vi "PropertyAdd.vi"(8 "error in":errorcluster, 11 "Data":T4) -> (0 "error out":errorcluster, 3 "Data 2":T4)   [LabVIEW 2017]
doc: "<B>This VI is used for adding a new property to the Caps file.</B>"
uses:
  Ctrl/Data.ctl
  Ctrl/Caps.ctl
  Ctrl/Property.ctl
  Ctrl/PhysicalChannel.ctl
  Ctrl/Register.ctl
  Ctrl/Bitfield.ctl
  Ctrl/Scale.ctl
  Ctrl/ScaleType.ctl
  Ctrl/Enum.ctl
  Ctrl/EnumValue.ctl
  Ctrl/Type Tab.ctl
  Ctrl/UserInput.ctl
  Ctrl/compond commands.ctl
panel:
  out "Data Range":T1
  in  "Min(Double)":dbl
  in  "Max(Double)":dbl
  in  "Max(U64)":u64
  in  "Min(U64)":u64
  in  "Min(I64)":i64
  in  "Max(I64)":i64
  in  "Max(U32)":u32
  in  "Min(U32)":u32
  in  "Min(I32)":i32
  in  "Max(I32)":i32
  in  "NewPropertyParameter:":T2 {"Value_Cluster"."U8" format="%.0x"; "Value_Cluster"."Ring" items=["False", "True"]; "Value_Cluster"."DBL" format="%#_16g"; "Scale" items=["NoScale"]; "Access" items=["Read Only", "Write Only", "Read/Write"]; "Bitfield" items=["Version/Timestamp", "TemperatureThreshold/TempThrehold", "TemperatureRegister3/AcquiredTemperature", "TemperatureRegister1/AcquiredTemperature", "TemperatureRegister2/AcquiredTemperature", "TemperatureRegister0/AcquiredTemperature", "Status/FlashWriteProtect", "Status/FlashHold", "Status/ClearWriteDuringUpdateError", "Status/SlscInterfaceUnusedPin", "Status/StrapOption", "Status/PowerGood5V", "Status/PowerGood24V", "Status/BoardFault", "Status/WriteDuringUpdateError", "Status/UpdateDone", "ClearFaults/OverTemperatureDigital", "ClearFaults/OverTemperature", "ClearFaults/OverCurrentOnBus", "ClearFaults/OverCurrentLow", "ClearFaults/OverCurrentHigh", "DigitalTempertureFault/TempFaultVector", "OverTemperature/OvertemperatureDifferential", "OverTemperature/OvertemperatureChannel", "OvercurrentLowStatus/OvercurrentLow", "OvercurrentHighStatus/OvercurrentHigh", "OvercurrentOnBus/BusB_OverCurrent", "OvercurrentOnBus/BusA_OverCurrent", "UpdateRegister/Update", "BoardControl/UpdateModeField", "BoardControl/BoardEnable", "BoardControl/TempSensorEnable", "StateRegister7/ChannelConnect", "StateRegister7/BusSelectionM", "StateRegister7/LoadEnableM", "StateRegister7/BusSelectionP", "StateRegister7/LoadEnableP", "PreloadRegister7/ChannelConnect", "PreloadRegister7/BusSelectionM", "PreloadRegister7/LoadEnableM", "PreloadRegister7/BusSelectionP", "PreloadRegister7/LoadEnableP", "StateRegister6/ChannelConnect", "StateRegister6/BusSelectionM", "StateRegister6/LoadEnableM", "StateRegister6/BusSelectionP", "StateRegister6/LoadEnableP", "PreloadRegister6/ChannelConnect", "PreloadRegister6/BusSelectionM", "PreloadRegister6/LoadEnableM", "PreloadRegister6/BusSelectionP", "PreloadRegister6/LoadEnableP", "StateRegister5/ChannelConnect", "StateRegister5/BusSelectionM", "StateRegister5/LoadEnableM", "StateRegister5/BusSelectionP", "StateRegister5/LoadEnableP", "PreloadRegister5/ChannelConnect", "PreloadRegister5/BusSelectionM", "PreloadRegister5/LoadEnableM", "PreloadRegister5/BusSelectionP", "PreloadRegister5/LoadEnableP", "StateRegister4/ChannelConnect", "StateRegister4/BusSelectionM", "StateRegister4/LoadEnableM", "StateRegister4/BusSelectionP", "StateRegister4/LoadEnableP", "PreloadRegister4/ChannelConnect", "PreloadRegister4/BusSelectionM", "PreloadRegister4/LoadEnableM", "PreloadRegister4/BusSelectionP", "PreloadRegister4/LoadEnableP", "StateRegister3/ChannelConnect", "StateRegister3/BusSelectionM", "StateRegister3/LoadEnableM", "StateRegister3/BusSelectionP", "StateRegister3/LoadEnableP", "PreloadRegister3/ChannelConnect", "PreloadRegister3/BusSelectionM", "PreloadRegister3/LoadEnableM", "PreloadRegister3/BusSelectionP", "PreloadRegister3/LoadEnableP", "StateRegister2/ChannelConnect", "StateRegister2/BusSelectionM", "StateRegister2/LoadEnableM", "StateRegister2/BusSelectionP", "StateRegister2/LoadEnableP", "PreloadRegister2/ChannelConnect", "PreloadRegister2/BusSelectionM", "PreloadRegister2/LoadEnableM", "PreloadRegister2/BusSelectionP", "PreloadRegister2/LoadEnableP", "StateRegister1/ChannelConnect", "StateRegister1/BusSelectionM", "StateRegister1/LoadEnableM", "StateRegister1/BusSelectionP", "StateRegister1/LoadEnableP", "PreloadRegister1/ChannelConnect", "PreloadRegister1/BusSelectionM", "PreloadRegister1/LoadEnableM", "PreloadRegister1/BusSelectionP", "PreloadRegister1/LoadEnableP", "StateRegister0/ChannelConnect", "StateRegister0/BusSelectionM", "StateRegister0/LoadEnableM", "StateRegister0/BusSelectionP", "StateRegister0/LoadEnableP", "PreloadRegister0/ChannelConnect", "PreloadRegister0/BusSelectionM", "PreloadRegister0/LoadEnableM", "PreloadRegister0/BusSelectionP", "PreloadRegister0/LoadEnableP", "SlowFilterCount/SlowCount", "FastFilterCount/FastCount", "SwitchDelayTime/CycleDelays", "InterruptAck/DigitalOverTemperatureIntAck", "InterruptAck/OverTemperatureIntAck", "InterruptAck/OverCurrentOnBusIntAck", "InterruptAck/OverCurrentLowIntAck", "InterruptAck/OverCurrentHighIntAck", "InterruptAck/UpdateDoneAck", "InterruptDisable/DigitalOverTemperatureIntDisable", "InterruptDisable/OverTemperatureIntDisable", "InterruptDisable/OverCurrentOnBusIntDisable", "InterruptDisable/OverCurrentLowIntDisable", "InterruptDisable/OverCurrentHighIntDisable", "InterruptDisable/UpdateDoneDisable", "InterruptEnable/DigitalOverTemperatureIntEnable", "InterruptEnable/OverTemperatureIntEnable", "InterruptEnable/OverCurrentOnBusIntEnable", "InterruptEnable/OverCurrentLowIntEnable", "InterruptEnable/OverCurrentHighIntEnable", "InterruptEnable/UpdateDoneEnable", "InterruptMask/DigitalOverTemperatureIntMask", "InterruptMask/OverTemperatureIntMask", "InterruptMask/OverCurrentOnBusIntMask", "InterruptMask/OverCurrentLowIntMask", "InterruptMask/OverCurrentHighIntMask", "InterruptMask/UpdateDoneMask", "InterruptStatus/DigitalOverTemperatureIntStatus", "InterruptStatus/OverTemperatureIntStatus", "InterruptStatus/OverCurrentOnBusIntStatus", "InterruptStatus/OverCurrentLowIntStatus", "InterruptStatus/OverCurrentHighIntStatus", "InterruptStatus/UpdateDone"]}
  out "CurrentAddPosition:":string="Current Adding Position:  NI.DateCode"
  in  "User Input":T3
  # "Value"
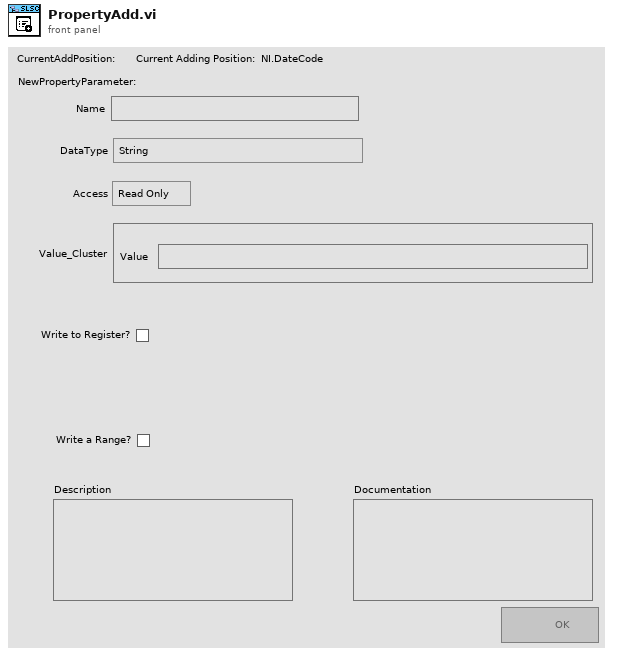
[diagram p1: front panel]
types:
  T1 = typedef "Type Tab.ctl" = enum32{"String", "Double", "U64", "I64", "U32", "I32", "Bool"}
  T2 = cluster{"Name":string, "DataType":enum16{"String", "Double", "U64", "I64", "U32", "I32", "Bool"}, "Bitfield":u16, "Access":u16, "Description":string, "Documentation":string, "OK Button":bool, "Scale":u16, "Write a Register?":bool, "Write a Range?":bool, "Value_Cluster":cluster{"DBL":dbl, "Ring":u16, "I64":i64, "U64":u64, "I32":i32, "U32":u32, "I8":i8, "U8":u8, "String":string}}
  T3 = typedef "UserInput.ctl" = cluster{"NewPropertyParameter":cluster{"Name":string, "DataType":enum16{"String", "Double", "U64", "I64", "U32", "I32", "Bool"}, "Bitfield":u16, "Access":u16, "Description":string, "Documentation":string, "OK Button":bool, "Scale method":u16, "Write a Register?":bool, "Write a Range?":bool, "Value_Cluster":cluster{"DBL":dbl, "Ring":u16, "I64":i64, "U64":u64, "I32":i32, "U32":u32, "I8":i8, "U8":u8, "String":string}}, "Min_Max_Cluster":cluster{"Min(Double)":dbl, "Max(Double)":dbl, "Min(U64)":u64, "Max(U64)":u64, "Min(I64)":i64, "Max(I64)":i64, "Min(U32)":u32, "Max(U32)":u32, "Min(I32)":i32, "Max(I32)":i32}, "Scale method":string, "Access":string, "Bitfield":string}
  T4 = typedef "Data.ctl" = cluster{"Ref Cluster":cluster{"String":refnum<vi>, "U8":refnum<vi>, "I8":refnum<vi>, "U32":refnum<vi>, "I32":refnum<vi>, "U64":refnum<vi>, "I64":refnum<vi>, "Ring":refnum<vi>, "DBL":refnum<vi>, "Add":refnum<vi>, "Remove":refnum<vi>, "Property tree":refnum<vi>, "confirm":refnum<vi>}, "JSON Text":string, "Original JSON Text":string, "Caps":T5, "SLSC Output Tree":cluster{"Left Cell String":string, "Child Text":string[], "Child Tag":string, "Item Indent":i32, "Child Only?":bool, "Glyph Index":i32, "offline value":variant}[], "Ref Index and Control Type":cluster{"index":i32, "Datatype":string}, "Selected Type and name":cluster{"Selected Type":enum16{"Property", "Physical Channel", "Other"}, "Selected Property Name":string}, "Update whole Tree?":bool}
  T5 = typedef "Caps.ctl" = cluster{"properties":T6[], "physical channels":T7[], "registers":T8[], "scales":T10[], "enums":T12[], "productName":string}
  T6 = typedef "Property.ctl" = cluster{"name":string, "bitfield":string, "value":variant, "dataType":string, "min":variant, "max":variant, "scale":string, "access":string}
  T7 = typedef "PhysicalChannel.ctl" = cluster{"name":string, "properties":T6[]}
  T8 = typedef "Register.ctl" = cluster{"name":string, "address":i32, "size":i32, "bitfields":T9[], "initialValue":variant, "connectedProperties":string[]}
  T9 = typedef "Bitfield.ctl" = cluster{"name":string, "offset":i32, "size":i32, "signed":bool}
  T10 = typedef "Scale.ctl" = cluster{"name":string, "type":T11, "params":variant}
  T11 = typedef "ScaleType.ctl" = enum16{"NoScale", "Table", "Polynomial", "Linear"}
  T12 = typedef "Enum.ctl" = cluster{"name":string, "values":T13[]}
  T13 = typedef "EnumValue.ctl" = cluster{"name":string, "value":i32}
  T14 = cluster{"Min(Double)":dbl, "Max(Double)":dbl, "Min(U64)":u64, "Max(U64)":u64, "Min(I64)":i64, "Max(I64)":i64, "Min(U32)":u32, "Max(U32)":u32, "Min(I32)":i32, "Max(I32)":i32}
  T15 = enum16{"String", "Double", "U64", "I64", "U32", "I32", "Bool"}
  T16 = enum8{"Enabled", "Disabled", "Disabled and Grayed Out"}
  T17 = cluster{"Name":string, "DataType":enum16{"String", "Double", "U64", "I64", "U32", "I32", "Bool"}, "Bitfield":u16, "Access":u16, "Description":string, "Documentation":string, "OK Button":bool, "Scale method":u16, "Write a Register?":bool, "Write a Range?":bool, "Value_Cluster":cluster{"DBL":dbl, "Ring":u16, "I64":i64, "U64":u64, "I32":i32, "U32":u32, "I8":i8, "U8":u8, "String":string}}
  T18 = cluster{"Duplicated?":bool, "InRange?":bool, "IsEmpty?":bool}
  T19 = typedef "compond commands.ctl" = enum16{"Get Property Array", "Get Physical Channel Property Array", "Get the Selected Position", "Get Property and Physical Channel Name", "Get Type and Value", "Make and Set a new Property", "Modify the Value", "Delete a Property"}
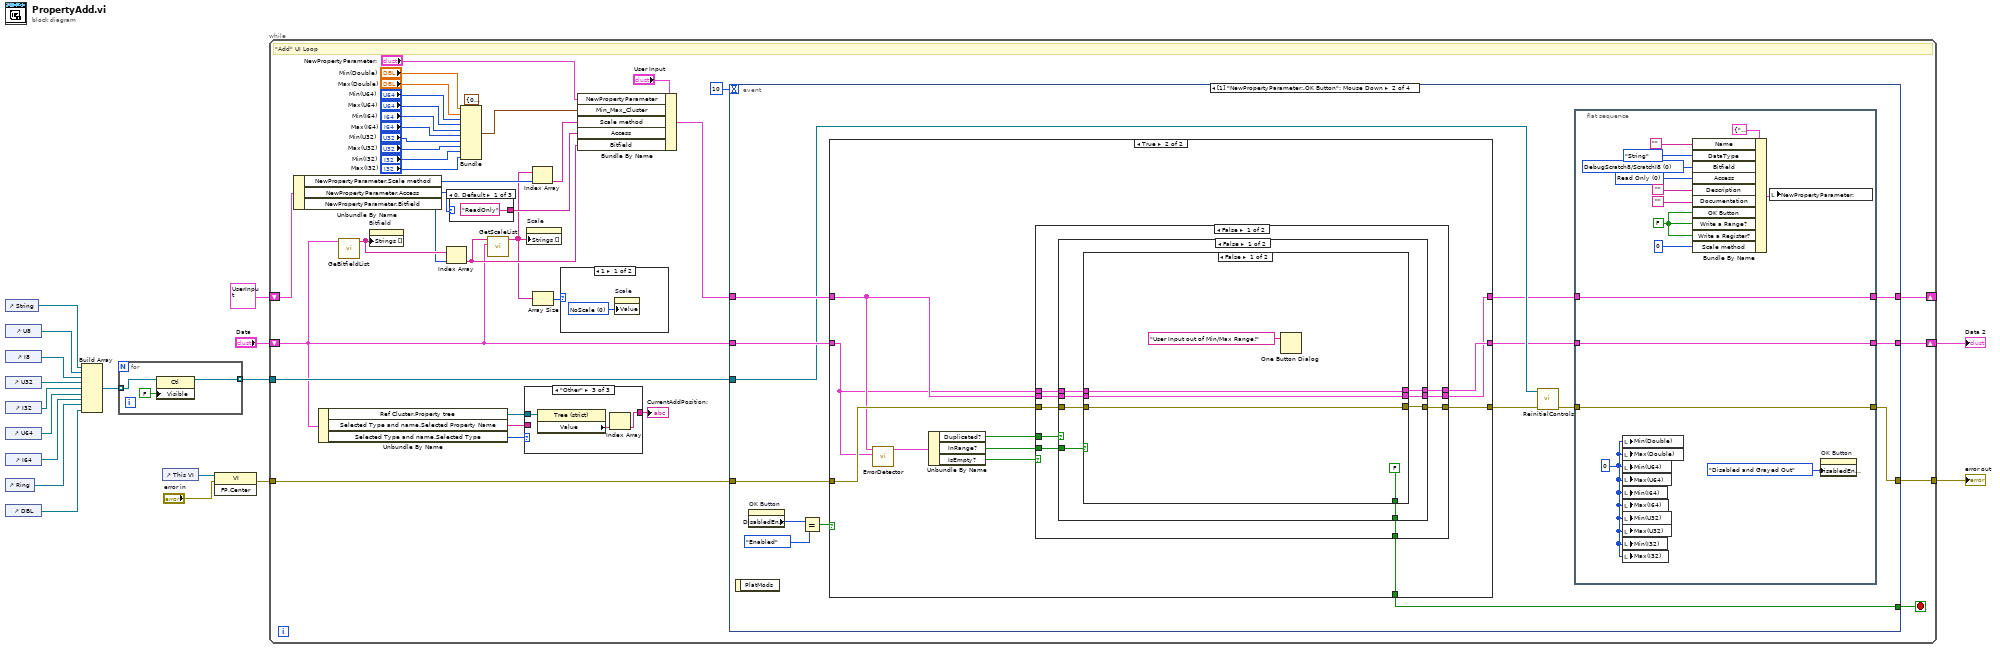
[diagram p0: block diagram]
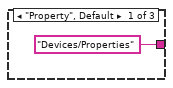
[diagram p2: hidden frame]
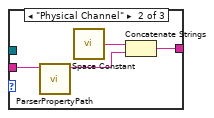
[diagram p3: hidden frame]
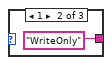
[diagram p5: hidden frame]
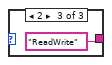
[diagram p6: hidden frame]
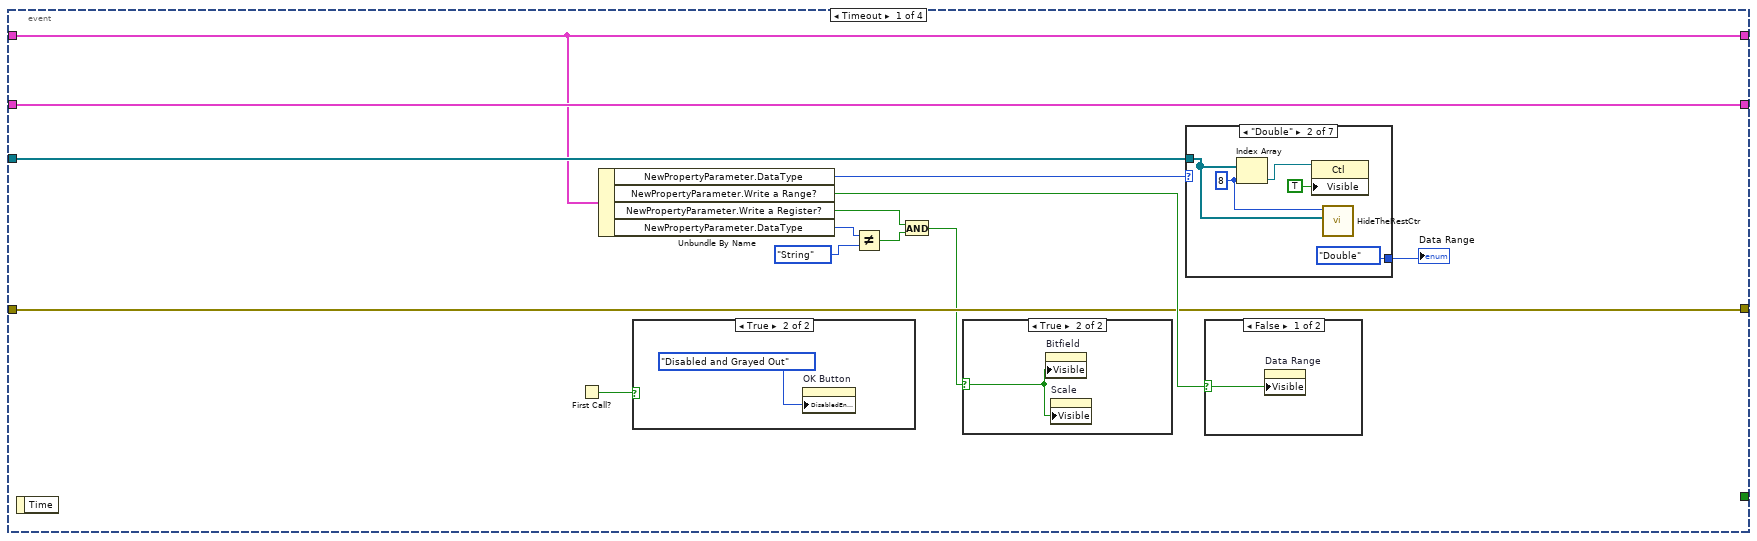
[diagram p7: hidden frame]
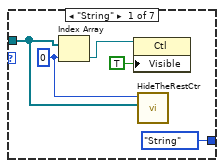
[diagram p8: hidden frame]
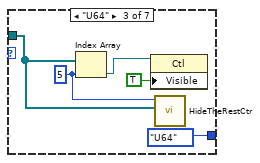
[diagram p9: hidden frame]
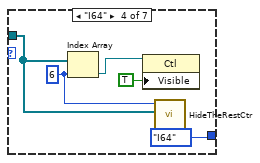
[diagram p10: hidden frame]
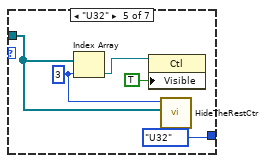
[diagram p11: hidden frame]
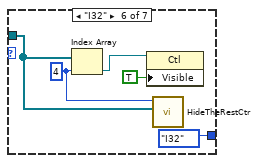
[diagram p12: hidden frame]
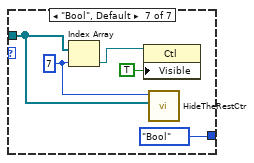
[diagram p13: hidden frame]
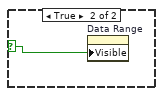
[diagram p14: hidden frame]
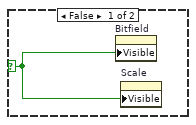
[diagram p15: hidden frame]
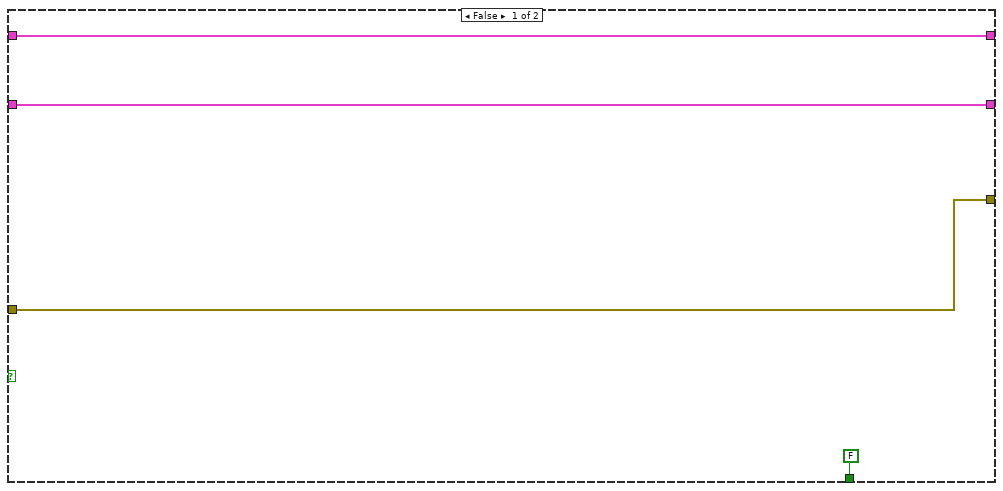
[diagram p17: hidden frame]
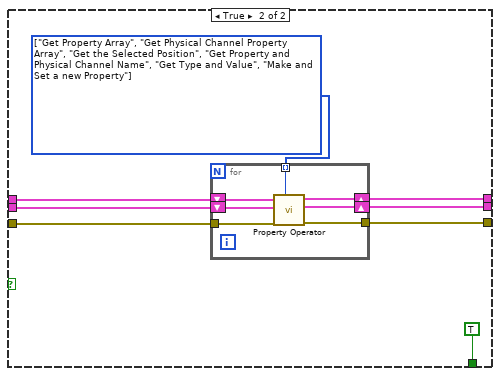
[diagram p18: hidden frame]
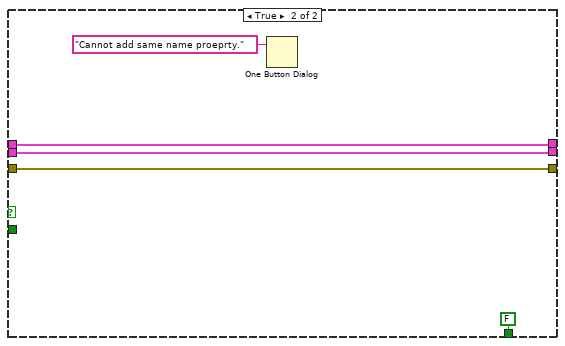
[diagram p19: hidden frame]
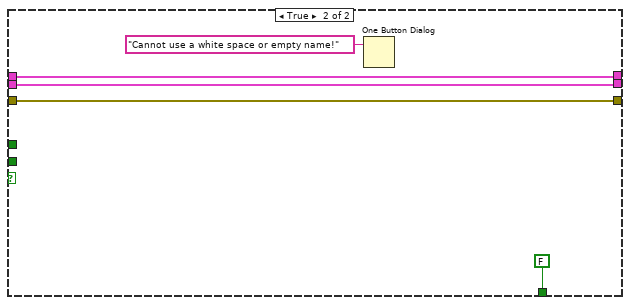
[diagram p20: hidden frame]
diagram:
  n1 = control-ref of="String"() -> (w18:refnum<vi>)
  n2 = control-ref of="U8"() -> (w17:refnum<vi>)
  n3 = control-ref of="I8"() -> (w16:refnum<vi>)
  n4 = control-ref of="U32"() -> (w15:refnum<vi>)
  n5 = control-ref of="I32"() -> (w14:refnum<vi>)
  n6 = control-ref of="U64"() -> (w13:refnum<vi>)
  n7 = control-ref of="I64"() -> (w12:refnum<vi>)
  n8 = control-ref of="Ring"() -> (w11:refnum<vi>)
  n9 = control-ref of="DBL"() -> (w10:refnum<vi>)
  n10 = Build Array(w18, w17, w16, w15, w14, w13, w12, w11, w10) -> (w3:refnum<vi>[])
  n11 = for {
    tunnel: w3 -> [w21] mode=indexing
    tunnel: [w19] -> w2 mode=indexing
    n12 = property class="Ctl"(reference=w21, "Visible"=FALSE) -> (reference out=w19:refnum<vi>)  [unwired: 1 in, 1 out]
  }
  n13 = control-ref of="This VI"() -> (w6:refnum<vi>)
  n14 = invoke class="VI" method="FP.Center"(reference=w6, error in="error in") -> (error out=w5:errorcluster)  [unwired: 1 in, 2 out]
  n15 = while {
    tunnel: w5 -> [w53]
    tunnel: [w57] -> w9
    shift-right: [w58] -> w7
    shift-left: "Data" -> [w26]
    shift-right: [w30] -> _
    shift-left: T3 {"NewPropertyParameter"={"Name"="", "DataType"=enum."String", "Bitfield"=0, "Access"=0, "Description"="", "Documentation"="", "OK Button"=FALSE, "Scale method"=0, "Write a Register?"=FALSE, "Write a Range?"=FALSE, "Value_Cluster"={"DBL"=0.0, "Ring"=0, "I64"=0, "U64"=0, "I32"=0, "U32"=0, "I8"=0, "U8"=0, "String"=""}}, "Min_Max_Cluster"={"Min(Double)"=0.0, "Max(Double)"=0.0, "Min(U64)"=0, "Max(U64)"=0, "Min(I64)"=0, "Max(I64)"=0, "Min(U32)"=0, "Max(U32)"=0, "Min(I32)"=0, "Max(I32)"=0}, "Scale method"="", "Access"="", "Bitfield"=""} ("User Input") -> [w40]
    tunnel: w2 -> [w31]
    stop <- w54 stop-if-true
    # "\"Add\" UI Loop"
    n16 = Unbundle By Name(w40) -> ("NewPropertyParameter.Scale method"=w36:u16, "NewPropertyParameter.Access"=w37:u16, "NewPropertyParameter.Bitfield"=w38:u16)
    n17 = Unbundle By Name(w26) -> ("Ref Cluster.Property tree"=w23:refnum<vi>, "Selected Type and name.Selected Property Name"=w25:string, "Selected Type and name.Selected Type"=w24:enum16{"Property", "Physical Channel", "Other"})
    n18 = call "GeBitfieldList.vi"("Data"=w26) -> ("Array"=w39:string[])  [unwired: 10 in]
    n19 = property on="Bitfield" class="Ring (strict)"("Strings []"=w39) -> ()  [unwired: 2 in, 2 out]
    n20 = Index Array(array=w39, index=w38) -> (element=w34:string)
    n21 = case shown="0, Default" w37 {
      tunnel: ["ReadOnly" "WriteOnly" "ReadWrite"] -> w33
      frame 0, Default {
      }
      frame 1 {
      }
      frame 2 {
      }
    }
    n22 = Bundle(cluster=T14 {"Min(Double)"=0.0, "Max(Double)"=0.0, "Min(U64)"=0, "Max(U64)"=0, "Min(I64)"=0, "Max(I64)"=0, "Min(U32)"=0, "Max(U32)"=0, "Min(I32)"=0, "Max(I32)"=0} ("Min_Max_Cluster"), "Min(Double)"="Min(Double)", "Max(Double)"="Max(Double)", "Min(U64)"="Min(U64)", "Max(U64)"="Max(U64)", "Min(I64)"="Min(I64)", "Max(I64)"="Max(I64)", "Min(U32)"="Min(U32)", "Max(U32)"="Max(U32)", "Min(I32)"="Min(I32)", "Max(I32)"="Max(I32)") -> (w52:T14)
    n23 = call "GetScaleList.vi"("Data in"=w26, "Bitfield in"=w34) -> ("output array"=w32:string[])  [unwired: 9 in]
    n24 = case shown="\"Other\"" w24 {
      tunnel: ["Devices/Properties" w63 w64] -> w28
      tunnel: w25 -> [_ w61 _]
      tunnel: w23 -> [_ _ w66]
      frame "Property", Default {
      }
      frame "Physical Channel" {
        n25 = call "ParserPropertyPath.vi"("Seleted Item Name"=w61) -> ("Physical channel"=w60:string)  [unwired: 7 in, 1 out]
        n26 = call <vilib>:"Space Constant.vi"() -> ("String"=w62:string)
        n27 = Concatenate Strings(w62, w60) -> (w63:string)
      }
      frame "Other" {
        n28 = property class="Tree (strict)"(reference=w66) -> ("Value"=w65:string[])  [unwired: 1 in, 2 out]
        n29 = Index Array(array=w65) -> (element=w64:string)  [unwired: 1 in]
      }
    }
    "CurrentAddPosition:" <- w28
    n30 = property on="Scale" class="Ring (strict)"("Strings []"=w32) -> ()  [unwired: 2 in, 2 out]
    n31 = Index Array(array=w32, index=w36) -> (element=w35:string)
    n32 = Array Size(array=w32) -> (size(s)=w55:i32)
    n33 = case shown="1" w55 {
      frame 1 {
        w67 = u16 0 items=["NoScale"] ("Scale method")
        n34 = property on="Scale" class="Ring (strict)"("Value"=w67) -> ()  [unwired: 2 in, 2 out]
      }
      frame Default {
      }
    }
    n35 = Bundle By Name(cluster="User Input", "NewPropertyParameter"="NewPropertyParameter:", "Min_Max_Cluster"=w52, "Scale method"=w35, "Access"=w33, "Bitfield"=w34) -> (w27:T3)
    n36 = event shown="[1] \"NewPropertyParameter:.OK Button\": Mouse Down" {
      selector: _ -> [_ _ _ _]
      dyn-events: _ -> [_ _ _ _]
      timeout: 10 -> [_ _ _ _]
      tunnel: w26 -> [w81 w138 w219 w236]
      tunnel: [w81 w127 w219 w236] -> w58
      tunnel: [w77 w124 w216 w235] -> w57
      tunnel: [_ w133 _ TRUE] -> w54
      tunnel: w53 -> [w77 w132 w216 w232]
      tunnel: w31 -> [w78 w130 _ w231]
      tunnel: w27 -> [w76 w131 w217 w230]
      tunnel: [w76 w125 w217 w230] -> w30
      event Timeout {
        n37 = event-data() -> ()  [unwired: 1 in, 1 out]
        n38 = First Call?() -> (First Call?: T/F=w82:bool)
        n39 = Unbundle By Name(w76) -> ("NewPropertyParameter.DataType"=w80:T15, "NewPropertyParameter.Write a Range?"=w79:bool, "NewPropertyParameter.Write a Register?"=w72:bool, "NewPropertyParameter.DataType"=w75:T15)
        n40 = case shown="True" w82 {
          frame False {
          }
          frame True {
            n41 = property on="OK Button" class="Bool (strict)"("DisabledEnum"=T16."Disabled and Grayed Out" ("Disabled")) -> ()  [unwired: 2 in, 2 out]
          }
        }
        n42 = Not Equal?(x=w75, y=T15."String") -> (x != y?=w73:bool)
        n43 = And(x=w72, y=w73) -> (x .and. y?=w71:bool)
        n44 = case shown="True" w71 {
          selector: w71 -> [w121 w122]
          frame False {
            n45 = property on="Bitfield" class="Ring (strict)"("Visible"=w121) -> ()  [unwired: 2 in, 2 out]
            n46 = property on="Scale" class="Ring (strict)"("Visible"=w121) -> ()  [unwired: 2 in, 2 out]
          }
          frame True {
            n47 = property on="Bitfield" class="Ring (strict)"("Visible"=w122) -> ()  [unwired: 2 in, 2 out]
            n48 = property on="Scale" class="Ring (strict)"("Visible"=w122) -> ()  [unwired: 2 in, 2 out]
          }
        }
        n49 = case shown="\"Double\"" w80 {
          tunnel: [Type_Tab."String" ("Tab Control") Type_Tab."Double" ("Tab Control") Type_Tab."U64" ("Tab Control") Type_Tab."I64" ("Tab Control") Type_Tab."U32" ("Tab Control") Type_Tab."I32" ("Tab Control") Type_Tab."Bool" ("Tab Control")] -> w83
          tunnel: w78 -> [w84 w89 w94 w99 w104 w109 w114]
          frame "String" {
            w87 = 0 ("index")
            n50 = Index Array(array=w84, index=w87) -> (element=w85:refnum<vi>)
            n51 = property class="Ctl"(reference=w85, "Visible"=TRUE) -> ()  [unwired: 1 in, 2 out]
            n52 = call "HideTheRestCtr.vi"("Array"=w84, "index"=w87) -> ()  [unwired: 10 in]
          }
          frame "Double" {
            w92 = 8 ("index")
            n53 = Index Array(array=w89, index=w92) -> (element=w90:refnum<vi>)
            n54 = property class="Ctl"(reference=w90, "Visible"=TRUE) -> ()  [unwired: 1 in, 2 out]
            n55 = call "HideTheRestCtr.vi"("Array"=w89, "index"=w92) -> ()  [unwired: 10 in]
          }
          frame "U64" {
            w97 = 5 ("index")
            n56 = Index Array(array=w94, index=w97) -> (element=w95:refnum<vi>)
            n57 = property class="Ctl"(reference=w95, "Visible"=TRUE) -> ()  [unwired: 1 in, 2 out]
            n58 = call "HideTheRestCtr.vi"("Array"=w94, "index"=w97) -> ()  [unwired: 10 in]
          }
          frame "I64" {
            w102 = 6 ("index")
            n59 = Index Array(array=w99, index=w102) -> (element=w100:refnum<vi>)
            n60 = property class="Ctl"(reference=w100, "Visible"=TRUE) -> ()  [unwired: 1 in, 2 out]
            n61 = call "HideTheRestCtr.vi"("Array"=w99, "index"=w102) -> ()  [unwired: 10 in]
          }
          frame "U32" {
            w107 = 3 ("index")
            n62 = Index Array(array=w104, index=w107) -> (element=w105:refnum<vi>)
            n63 = property class="Ctl"(reference=w105, "Visible"=TRUE) -> ()  [unwired: 1 in, 2 out]
            n64 = call "HideTheRestCtr.vi"("Array"=w104, "index"=w107) -> ()  [unwired: 10 in]
          }
          frame "I32" {
            w112 = 4 ("index")
            n65 = Index Array(array=w109, index=w112) -> (element=w110:refnum<vi>)
            n66 = property class="Ctl"(reference=w110, "Visible"=TRUE) -> ()  [unwired: 1 in, 2 out]
            n67 = call "HideTheRestCtr.vi"("Array"=w109, "index"=w112) -> ()  [unwired: 10 in]
          }
          frame "Bool", Default {
            w117 = 7 ("index")
            n68 = Index Array(array=w114, index=w117) -> (element=w115:refnum<vi>)
            n69 = property class="Ctl"(reference=w115, "Visible"=TRUE) -> ()  [unwired: 1 in, 2 out]
            n70 = call "HideTheRestCtr.vi"("Array"=w114, "index"=w117) -> ()  [unwired: 10 in]
          }
        }
        "Data Range" <- w83
        n71 = case shown="False" w79 {
          selector: w79 -> [w119 w120]
          frame False {
            n72 = property on="Data Range" class="TabCtl (strict)"("Visible"=w119) -> ()  [unwired: 2 in, 2 out]
          }
          frame True {
            n73 = property on="Data Range" class="TabCtl (strict)"("Visible"=w120) -> ()  [unwired: 2 in, 2 out]
          }
        }
      }
      event "NewPropertyParameter:.OK Button": Mouse Down {
        n74 = event-data() -> ()  [unwired: 1 in, 1 out]
        n75 = property on="OK Button" class="Bool (strict)"() -> ("DisabledEnum"=w135:T16)  [unwired: 2 in, 2 out]
        n76 = Equal?(x=w135, y=T16."Enabled") -> (x = y?=w136:bool)
        n77 = case shown="True" w136 {
          tunnel: w138 -> [w157 w162]
          tunnel: [w157 w167] -> w128
          tunnel: [w155 w166] -> w137
          tunnel: [FALSE w168] -> w133
          tunnel: w131 -> [w154 w163]
          tunnel: w132 -> [w155 w165]
          tunnel: [w154 w164] -> w126
          frame False {
          }
          frame True {
            n78 = call "ErrorDetector.vi"("Data"=w162, "User Input"=w163) -> ("Cluster"=w161:T18)  [unwired: 9 in]
            n79 = Unbundle By Name(w161) -> ("Duplicated?"=w160:bool, "InRange?"=w159:bool, "IsEmpty?"=w158:bool)
            n80 = case shown="False" w158 {
              tunnel: [w177 FALSE] -> w168
              tunnel: [w176 w213] -> w167
              tunnel: [w175 w214] -> w166
              tunnel: w165 -> [w174 w214]
              tunnel: [w173 w212] -> w164
              tunnel: w160 -> [w172 _]
              tunnel: w162 -> [w171 w213]
              tunnel: w159 -> [w170 _]
              tunnel: w163 -> [w169 w212]
              frame False {
                n81 = case shown="False" w172 {
                  tunnel: [w185 FALSE] -> w177
                  tunnel: [w184 w210] -> w176
                  tunnel: [w183 w208] -> w175
                  tunnel: w174 -> [w182 w208]
                  tunnel: [w181 w209] -> w173
                  tunnel: w169 -> [w180 w209]
                  tunnel: w171 -> [w179 w210]
                  tunnel: w170 -> [w178 _]
                  frame False {
                    n82 = case shown="False" w178 {
                      tunnel: [FALSE TRUE] -> w185
                      tunnel: w179 -> [w190 w197]
                      tunnel: [w190 w196] -> w184
                      tunnel: w180 -> [w189 w195]
                      tunnel: [w189 w194] -> w181
                      tunnel: w182 -> [w188 w193]
                      tunnel: [w188 w192] -> w183
                      frame False {
                        n83 = One Button Dialog(message="User Input out of Min/Max Range!") -> ()  [unwired: 1 in, 1 out]
                      }
                      frame True {
                        w191 = T19[] [enum."Get Property Array", enum."Get Physical Channel Property Array", enum."Get the Selected Position", enum."Get Property and Physical Channel Name", enum."Get Type and Value", enum."Make and Set a new Property"] items=["Get Property Array", "Get Physical Channel Property Array", "Get the Selected Position", "Get Property and Physical Channel Name", "Get Type and Value", "Make and Set a new Property", "Modify the Value", "Delete a Property"]
                        n84 = for {
                          tunnel: w193 -> [w201]
                          tunnel: [w200] -> w192
                          shift-right: [w204] -> w196
                          shift-left: w197 -> [w205]
                          shift-right: [w202] -> w194
                          shift-left: w195 -> [w203]
                          tunnel: w191 -> [w199] mode=indexing
                          n85 = call "Property Operator.vi"("Command"=w199, "error in"=w201, "User Input"=w203, "Data Input"=w205) -> ("error out"=w200:errorcluster, "User Input 2"=w202:T3, "Data Output"=w204:T4)  [unwired: 5 in]
                        }
                      }
                    }
                  }
                  frame True {
                    n86 = One Button Dialog(message="Cannot add same name proeprty.") -> ()  [unwired: 1 in, 1 out]
                  }
                }
              }
              frame True {
                n87 = One Button Dialog(message="Cannot use a white space or empty name!") -> ()  [unwired: 1 in, 1 out]
              }
            }
          }
        }
        n88 = call "ReinitialControls.vi"("error in (no error)"=w137, "Control reference Array"=w130) -> ("error out"=w129:errorcluster)  [unwired: 9 in]
        n89 = flat-sequence {
          tunnel: w129 -> [w144]
          tunnel: [w144] -> w124
          tunnel: w128 -> [w143]
          tunnel: [w143] -> w127
          tunnel: [w142] -> w125
          tunnel: w126 -> [w142]
          frame #0 {
            w141 = FALSE ("OK Button")
            w147 = u16 0 items=["Read Only", "Write Only", "Read/Write"] ("Access")
            w148 = u16 0 items=["DebugScratch8/ScratchI8", "DebugScratch8/Scratch8", "DebugScratch8/ScratchBool", "DebugScratch16/ScratchBool", "DebugScratch16/ScratchI8", "DebugScratch16/Scratch8", "DebugScratch16/ScratchI16", "DebugScratch16/Scratch16", "DebugScratch32/ScratchBool", "DebugScratch32/ScratchI8", "DebugScratch32/Scratch8", "DebugScratch32/ScratchI16", "DebugScratch32/Scratch16", "DebugScratch32/ScratchI32", "DebugScratch32/Scratch32", "DebugLeds/DebugLed3", "DebugLeds/DebugLed2", "DebugLeds/DebugLed1", "DebugLeds/DebugLed0", "DebugDipSwitch/DipSwitch8", "DebugDipSwitch/DipSwitch7", "DebugDipSwitch/DipSwitch6", "DebugDipSwitch/DipSwitch5", "DebugDipSwitch/DipSwitch4", "DebugDipSwitch/DipSwitch3", "DebugDipSwitch/DipSwitch2", "DebugDipSwitch/DipSwitch1", "DebugScratch64/ScratchBool", "DebugScratch64/ScratchI8", "DebugScratch64/Scratch8", "DebugScratch64/ScratchI16", "DebugScratch64/Scratch16", "DebugScratch64/ScratchI32", "DebugScratch64/Scratch32", "DebugScratch64/ScratchI64", "DebugScratch64/Scratch64", "FrontPanelLeds/LedRed0Enable", "FrontPanelLeds/LedRed1Enable", "FrontPanelLeds/LedRed2Enable", "FrontPanelLeds/LedGreen0Enable", "FrontPanelLeds/LedGreen1Enable", "FrontPanelLeds/LedGreen2Enable", "Revision/DateCode", "InterruptAck/EventIntAck0", "InterruptAck/EventIntAck1", "InterruptAck/EventIntAck2", "InterruptAck/EventIntAck3", "InterruptAck/ExternalIntAck0", "InterruptAck/ExternalIntAck1", "InterruptAck/ExternalIntAck2", "InterruptAck/ExternalIntAck3", "InterruptDisable/EventIntDisable0", "InterruptDisable/EventIntDisable1", "InterruptDisable/EventIntDisable2", "InterruptDisable/EventIntDisable3", "InterruptDisable/ExternalIntDisable0", "InterruptDisable/ExternalIntDisable1", "InterruptDisable/ExternalIntDisable2", "InterruptDisable/ExternalIntDisable3", "InterruptEnable/EventIntEnable0", "InterruptEnable/EventIntEnable1", "InterruptEnable/EventIntEnable2", "InterruptEnable/EventIntEnable3", "InterruptEnable/ExternalIntEnable0", "InterruptEnable/ExternalIntEnable1", "InterruptEnable/ExternalIntEnable2", "InterruptEnable/ExternalIntEnable3", "InterruptMask/EventIntMask0", "InterruptMask/EventIntMask1", "InterruptMask/EventIntMask2", "InterruptMask/EventIntMask3", "InterruptMask/ExternalIntMask0", "InterruptMask/ExternalIntMask1", "InterruptMask/ExternalIntMask2", "InterruptMask/ExternalIntMask3", "InterruptStatus/EventIntStatus0", "InterruptStatus/EventIntStatus1", "InterruptStatus/EventIntStatus2", "InterruptStatus/EventIntStatus3", "InterruptStatus/ExternalIntStatus0", "InterruptStatus/ExternalIntStatus1", "InterruptStatus/ExternalIntStatus2", "InterruptStatus/ExternalIntStatus3", "EventCounter3/DelayInMilliseconds", "EventCounter2/DelayInMilliseconds", "EventCounter1/DelayInMilliseconds", "EventCounter0/DelayInMilliseconds", "EventStartRegister/EventStart0", "EventStartRegister/EventStart1", "EventStartRegister/EventStart2", "EventStartRegister/EventStart3"] ("Bitfield")
            w153 = u64 0 ("Min(U64)")
            n90 = local write "Min(Double)"(w153) -> ()
            n91 = local write "Max(Double)"(w153) -> ()
            n92 = local write "Min(U64)"(w153) -> ()
            n93 = local write "Max(U64)"(w153) -> ()
            n94 = local write "Min(I64)"(w153) -> ()
            n95 = local write "Max(I64)"(w153) -> ()
            n96 = local write "Min(U32)"(w153) -> ()
            n97 = local write "Max(U32)"(w153) -> ()
            n98 = local write "Min(I32)"(w153) -> ()
            n99 = local write "Max(I32)"(w153) -> ()
            n100 = Bundle By Name(cluster=T17 {"Name"="abc", "DataType"=enum."Double", "Bitfield"=0, "Access"=1, "Description"="ab", "Documentation"="ab", "OK Button"=FALSE, "Scale method"=0, "Write a Register?"=FALSE, "Write a Range?"=TRUE, "Value_Cluster"={"DBL"=0.0, "Ring"=0, "I64"=0, "U64"=0, "I32"=0, "U32"=0, "I8"=0, "U8"=0, "String"=""}} ("NewPropertyParameter"), "Name"="", "DataType"=T15."String", "Bitfield"=w148, "Access"=w147, "Description"="", "Documentation"="", "OK Button"=w141, "Write a Range?"=w141, "Write a Register?"=w141, "Scale method"=u16 0) -> (w152:T17)
            n101 = local write "NewPropertyParameter:"(w152) -> ()
            n102 = property on="OK Button" class="Bool (strict)"("DisabledEnum"=T16."Disabled and Grayed Out" ("Disabled")) -> ()  [unwired: 2 in, 2 out]
          }
        }
      }
      event "NewPropertyParameter:.Name": Value Change {
        n103 = event-data() -> ()  [unwired: 1 in, 1 out]
        n104 = property on="OK Button" class="Bool (strict)"("DisabledEnum"=T16."Enabled" ("Disabled")) -> ()  [unwired: 2 in, 2 out]
      }
      event Panel Close {
        w221 = FALSE ("Write a Register?")
        w233 = u64 0 ("Min(U64)")
        w224 = u16 0 items=["Read Only", "Write Only", "Read/Write"] ("Access")
        w225 = u16 0 items=["DebugScratch8/ScratchI8", "DebugScratch8/Scratch8", "DebugScratch8/ScratchBool", "DebugScratch16/ScratchBool", "DebugScratch16/ScratchI8", "DebugScratch16/Scratch8", "DebugScratch16/ScratchI16", "DebugScratch16/Scratch16", "DebugScratch32/ScratchBool", "DebugScratch32/ScratchI8", "DebugScratch32/Scratch8", "DebugScratch32/ScratchI16", "DebugScratch32/Scratch16", "DebugScratch32/ScratchI32", "DebugScratch32/Scratch32", "DebugLeds/DebugLed3", "DebugLeds/DebugLed2", "DebugLeds/DebugLed1", "DebugLeds/DebugLed0", "DebugDipSwitch/DipSwitch8", "DebugDipSwitch/DipSwitch7", "DebugDipSwitch/DipSwitch6", "DebugDipSwitch/DipSwitch5", "DebugDipSwitch/DipSwitch4", "DebugDipSwitch/DipSwitch3", "DebugDipSwitch/DipSwitch2", "DebugDipSwitch/DipSwitch1", "DebugScratch64/ScratchBool", "DebugScratch64/ScratchI8", "DebugScratch64/Scratch8", "DebugScratch64/ScratchI16", "DebugScratch64/Scratch16", "DebugScratch64/ScratchI32", "DebugScratch64/Scratch32", "DebugScratch64/ScratchI64", "DebugScratch64/Scratch64", "FrontPanelLeds/LedRed0Enable", "FrontPanelLeds/LedRed1Enable", "FrontPanelLeds/LedRed2Enable", "FrontPanelLeds/LedGreen0Enable", "FrontPanelLeds/LedGreen1Enable", "FrontPanelLeds/LedGreen2Enable", "Revision/DateCode", "InterruptAck/EventIntAck0", "InterruptAck/EventIntAck1", "InterruptAck/EventIntAck2", "InterruptAck/EventIntAck3", "InterruptAck/ExternalIntAck0", "InterruptAck/ExternalIntAck1", "InterruptAck/ExternalIntAck2", "InterruptAck/ExternalIntAck3", "InterruptDisable/EventIntDisable0", "InterruptDisable/EventIntDisable1", "InterruptDisable/EventIntDisable2", "InterruptDisable/EventIntDisable3", "InterruptDisable/ExternalIntDisable0", "InterruptDisable/ExternalIntDisable1", "InterruptDisable/ExternalIntDisable2", "InterruptDisable/ExternalIntDisable3", "InterruptEnable/EventIntEnable0", "InterruptEnable/EventIntEnable1", "InterruptEnable/EventIntEnable2", "InterruptEnable/EventIntEnable3", "InterruptEnable/ExternalIntEnable0", "InterruptEnable/ExternalIntEnable1", "InterruptEnable/ExternalIntEnable2", "InterruptEnable/ExternalIntEnable3", "InterruptMask/EventIntMask0", "InterruptMask/EventIntMask1", "InterruptMask/EventIntMask2", "InterruptMask/EventIntMask3", "InterruptMask/ExternalIntMask0", "InterruptMask/ExternalIntMask1", "InterruptMask/ExternalIntMask2", "InterruptMask/ExternalIntMask3", "InterruptStatus/EventIntStatus0", "InterruptStatus/EventIntStatus1", "InterruptStatus/EventIntStatus2", "InterruptStatus/EventIntStatus3", "InterruptStatus/ExternalIntStatus0", "InterruptStatus/ExternalIntStatus1", "InterruptStatus/ExternalIntStatus2", "InterruptStatus/ExternalIntStatus3", "EventCounter3/DelayInMilliseconds", "EventCounter2/DelayInMilliseconds", "EventCounter1/DelayInMilliseconds", "EventCounter0/DelayInMilliseconds", "EventStartRegister/EventStart0", "EventStartRegister/EventStart1", "EventStartRegister/EventStart2", "EventStartRegister/EventStart3"] ("Bitfield")
        n105 = event-data() -> ()  [unwired: 1 in, 1 out]
        n106 = call "ReinitialControls.vi"("error in (no error)"=w232, "Control reference Array"=w231) -> ("error out"=w235:errorcluster)  [unwired: 9 in]
        n107 = local write "Min(Double)"(w233) -> ()
        n108 = local write "Max(Double)"(w233) -> ()
        n109 = local write "Min(U64)"(w233) -> ()
        n110 = local write "Max(U64)"(w233) -> ()
        n111 = local write "Min(I64)"(w233) -> ()
        n112 = local write "Max(I64)"(w233) -> ()
        n113 = local write "Min(U32)"(w233) -> ()
        n114 = local write "Max(U32)"(w233) -> ()
        n115 = local write "Min(I32)"(w233) -> ()
        n116 = local write "Max(I32)"(w233) -> ()
        n117 = Bundle By Name(cluster=T17 {"Name"="abc", "DataType"=enum."Double", "Bitfield"=0, "Access"=1, "Description"="ab", "Documentation"="ab", "OK Button"=FALSE, "Scale method"=0, "Write a Register?"=FALSE, "Write a Range?"=TRUE, "Value_Cluster"={"DBL"=0.0, "Ring"=0, "I64"=0, "U64"=0, "I32"=0, "U32"=0, "I8"=0, "U8"=0, "String"=""}} ("NewPropertyParameter"), "Name"="", "DataType"=T15."String", "Bitfield"=w225, "Access"=w224, "Description"="", "Documentation"="", "OK Button"=w221, "Scale method"=u16 0, "Write a Register?"=w221, "Write a Range?"=w221) -> (w228:T17)
        n118 = local write "NewPropertyParameter:"(w228) -> ()
      }
    }
  }
  "error out" <- w9
  "Data 2" <- w7
